vi "[ex ce] History of Script Variable.vi"() -> ()   [LabVIEW 2021]
doc: "<B>Variable Manager example</B>\n\nThe VI demonstrates details of how variable history works depending on its configuration. A variable is updated in CSE script and its history is read and indicated in parallel loop.\n\n::: CalcExpress Toolkit :::\nCopyright (c) 2000-2026 Konstantin Shifershteyn. All rights reserved."
uses:
  vi.lib/addons/CalcExpress/cetypes.llb/VarMan History Info.ctl
panel:
  in  "Value condition":T1 {"Range Max" format="%.3f"; "Range Min" format="%.3f"; "Delta" format="%.3f"}
  in  "Time condition":cluster{"Step, ms":i32, "Gate, ms":u32}
  in  "Condition selector":u16(ring)=1 caption="conditions example" items=["<custom condition>", "no conditions", "time step", "time step & out of range", "time step & time gate", "out of range", "within range"]
  out "graph":T2(graph) caption="The graph indicates history of the 'x' variable"
  out "history info":T3 caption="History info" {"oldest timestamp" format="%<%H:%M:%S%2u\n%d/%m/%Y>T"; "NewVals mode"."last read time" format="%<%H:%M:%S%2u\n%d/%m/%Y>T"; "newest timestamp" format="%<%H:%M:%S%2u\n%d/%m/%Y>T"}
  in  "History length":i32=100
  in  "script":string="if (x>=20) dx = -1;\nif (x<=0)  dx = 1;\nx += dx;\n"
  in  "stop":bool
  # "History Update Conditions"
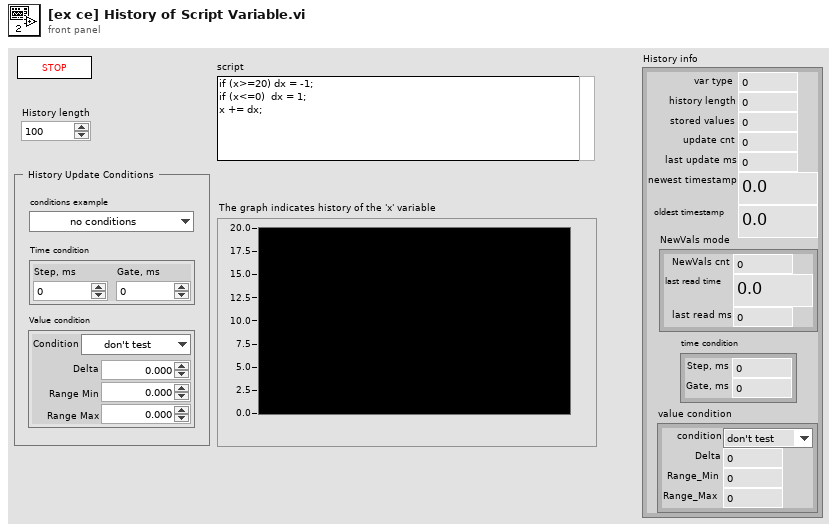
[diagram p1: front panel]
types:
  T1 = cluster{"Condition":enum32{"don't test", "changed", "abs deviation", "rel deviation", "out of range", "within range"}, "Delta":dbl, "Range Min":dbl, "Range Max":dbl}
  T2 = cluster{"history timestamps":dbl[], "history values":dbl[]}
  T3 = typedef "VarMan History Info.ctl" = cluster{"var type":u32, "history length":u32, "stored values":u32, "update cnt":u32, "last update ms":u32, "newest timestamp":dbl, "oldest timestamp":dbl, "NewVals mode":cluster{"NewVals cnt":u32, "last read time":dbl, "last read ms":u32}, "time condition":cluster{"Step, ms":u32, "Gate, ms":u32}, "value condition":cluster{"condition":enum32{"don't test", "changed", "abs deviation", "rel deviation", "out of range", "within range"}, "Delta":dbl, "Range_Min":dbl, "Range_Max":dbl}}
  T4 = cluster{"condition":enum32{"don't test", "changed", "abs deviation", "rel deviation", "out of range", "within range"}, "Delta":dbl, "Range_Min":dbl, "Range_Max":dbl}[]
  T5 = enum16{"create", "destroy", "set value", "get value"}
  T6 = enum32{"nop", "create", "destroy", "reset", "get info", "config"}
  T7 = typedef "VarMan Variable Context Handle.ctl" = i32
  T8 = cluster{"condition":enum32{"don't test", "changed", "abs deviation", "rel deviation", "out of range", "within range"}, "Delta":dbl, "Range_Min":dbl, "Range_Max":dbl}
  T9 = typedef "CSE Instance RefNum.ctl" = refnum<k1>
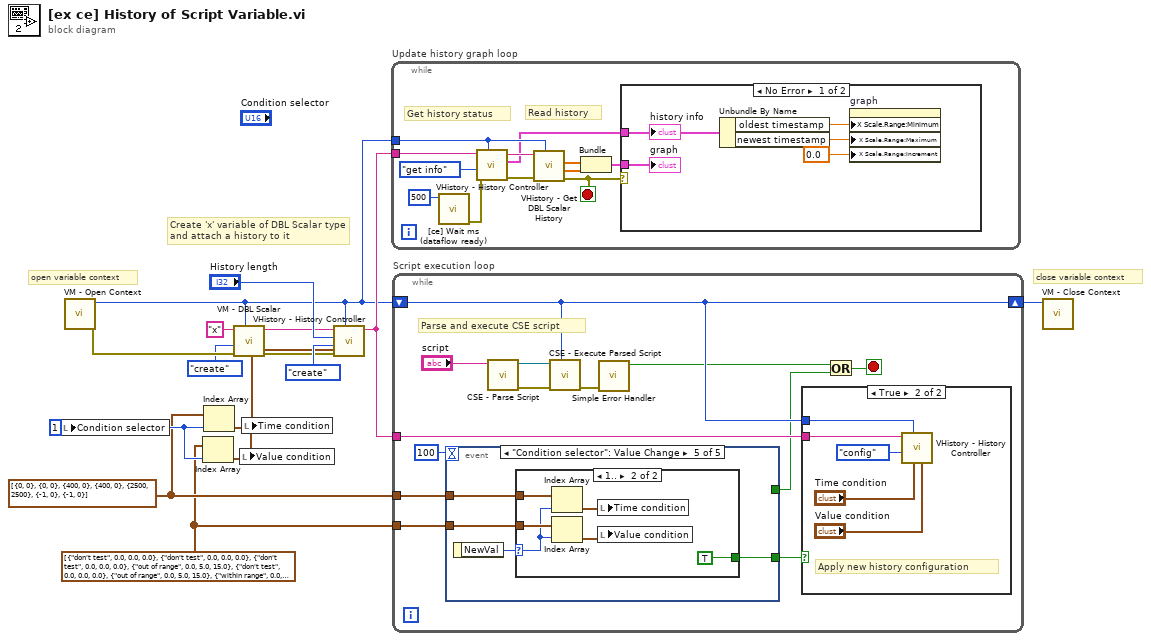
[diagram p0: block diagram]
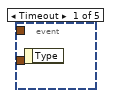
[diagram p2: hidden frame]
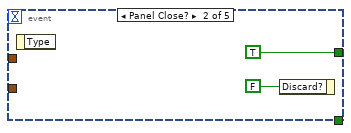
[diagram p3: hidden frame]
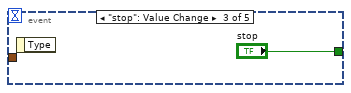
[diagram p4: hidden frame]
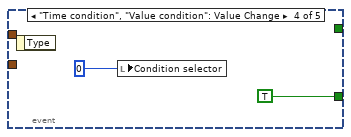
[diagram p5: hidden frame]
diagram:
  w5 = u16 1
  w1 = T4 [{"condition"=enum."don't test", "Delta"=0.0, "Range_Min"=0.0, "Range_Max"=0.0}, {"condition"=enum."don't test", "Delta"=0.0, "Range_Min"=0.0, "Range_Max"=0.0}, {"condition"=enum."don't test", "Delta"=0.0, "Range_Min"=0.0, "Range_Max"=0.0}, {"condition"=enum."out of range", "Delta"=0.0, "Range_Min"=5.0, "Range_Max"=15.0}, {"condition"=enum."don't test", "Delta"=0.0, "Range_Min"=0.0, "Range_Max"=0.0}, {"condition"=enum."out of range", "Delta"=0.0, "Range_Min"=5.0, "Range_Max"=15.0}, {"condition"=enum."within range", "Delta"=0.0, "Range_Min"=5.0, "Range_Max"=15.0}]
  w4 = cluster{"Step, ms":i32, "Gate, ms":u32}[] [{"Step, ms"=0, "Gate, ms"=0}, {"Step, ms"=0, "Gate, ms"=0}, {"Step, ms"=400, "Gate, ms"=0}, {"Step, ms"=400, "Gate, ms"=0}, {"Step, ms"=2500, "Gate, ms"=2500}, {"Step, ms"=-1, "Gate, ms"=0}, {"Step, ms"=-1, "Gate, ms"=0}]
  # "close variable context"
  # "Create 'x' variable of DBL Scalar type\nand attach a history to it"
  # "open variable context"
  n1 = local write "Condition selector"(w5) -> ()
  n2 = call "VM - Open Context.vi"() -> ("error out"=w11:errorcluster, "VC Handle out"=w6:T7)  [unwired: 9 in, 1 out]
  n3 = Index Array(array=w1, index=w5) -> (element=w2:T8)
  n4 = Index Array(array=w4, index=w5) -> (element=w3:cluster{"Step, ms":i32, "Gate, ms":u32})
  n5 = call "VM - DBL Scalar.vi"("VC Handle"=w6, "error in"=w11, "cmd"=T5."create", "name_spec"="x" ("name")) -> ("error out"=w12:errorcluster, "dup name_spec"=w8:string)  [unwired: 2 in, 4 out]
  n6 = local write "Value condition"(w2) -> ()
  n7 = local write "Time condition"(w3) -> ()
  n8 = call "VHistory - History Controller.vi"("value condition"=w2, "time conditions"=w3, "VC Handle"=w6, "error in"=w12, "cmd (nop:default)"=T6."create", "history length"="History length", "name_spec"=w8) -> ("dup name_spec"=w7:string)  [unwired: 1 in, 3 out]
  n9 = while "Update history graph loop" {
    tunnel: w6 -> [w21]
    tunnel: w7 -> [w22]
    stop <- w16 stop-if-true
    # "Read history"
    # "Get history status"
    n10 = call "[ce] Wait ms (dataflow ready).vi"("milliseconds to wait"=u32 500) -> ("error out"=w17:errorcluster)  [unwired: 4 in, 4 out]
    n11 = call "VHistory - History Controller.vi"("VC Handle"=w21, "error in"=w17, "cmd (nop:default)"=T6."get info", "name_spec"=w22) -> ("error out"=w24:errorcluster, "history info"=w20:T3, "dup name_spec"=w23:string)  [unwired: 4 in, 1 out]
    n12 = call "VHistory - Get DBL Scalar History.vi"("VC Handle"=w21, "error in"=w24, "name_spec"=w23) -> ("error out"=w16:errorcluster, "history"=w27:dbl[], "time stamps"=w25:dbl[])  [unwired: 4 in, 2 out]
    n13 = Bundle("time stamps"=w25, "history"=w27) -> (w26:cluster{"time stamps":dbl[], "history":dbl[]})  [unwired: 1 in]
    n14 = case shown="No Error" w16 {
      tunnel: w26 -> [w32 _]
      tunnel: w20 -> [w31 _]
      frame No Error {
        n15 = Unbundle By Name(w31) -> ("oldest timestamp"=w30:dbl, "newest timestamp"=w29:dbl)
        n16 = property on="graph" class="XYGraph (strict)"("X Scale.Range:Minimum"=w30, "X Scale.Range:Maximum"=w29, "X Scale.Range:Increment"=0.0 ("X Increment")) -> ()  [unwired: 2 in, 2 out]
        "graph" <- w32
        "history info" <- w31
      }
      frame Error {
      }
    }
  }
  n17 = while "Script execution loop" {
    tunnel: w1 -> [w37]
    tunnel: w4 -> [w38]
    tunnel: w7 -> [w42]
    shift-left: w6 -> [w41]
    shift-right: [w41] -> w15
    stop <- w33 stop-if-true
    # "Parse and execute CSE script"
    n18 = event shown="[4] \"Condition selector\": Value Change" {
      selector: _ -> [_ _ _ _ _]
      dyn-events: _ -> [_ _ _ _ _]
      timeout: 100 -> [_ _ _ _ _]
      tunnel: w38 -> [_ _ _ _ w54]
      tunnel: w37 -> [_ _ _ _ w53]
      tunnel: [_ _ _ TRUE w51] -> w36
      tunnel: [_ TRUE "stop" _ _] -> w35
      event Timeout {
        n19 = event-data() -> ()  [unwired: 1 in, 1 out]
      }
      event Panel Close? {
        n20 = event-data() -> ()  [unwired: 1 in, 1 out]
        n21 = event-data("Discard?"=FALSE) -> ()  [unwired: 1 in, 1 out]
      }
      event "stop": Value Change {
        n22 = event-data() -> ()  [unwired: 1 in, 1 out]
      }
      event "Time condition", "Value condition": Value Change {
        n23 = event-data() -> ()  [unwired: 1 in, 1 out]
        n24 = local write "Condition selector"(u16 0) -> ()
      }
      event "Condition selector": Value Change {
        n25 = event-data() -> ("NewVal"=w52:u16)  [unwired: 1 in]
        n26 = case shown="1.." w52 {
          selector: w52 -> [_ w56]
          tunnel: w54 -> [_ w58]
          tunnel: w53 -> [_ w57]
          tunnel: [_ TRUE] -> w51
          frame ..0 {
          }
          frame 1.. {
            n27 = Index Array(array=w58, index=w56) -> (element=w59:cluster{"Step, ms":i32, "Gate, ms":u32})
            n28 = Index Array(array=w57, index=w56) -> (element=w60:T8)
            n29 = local write "Time condition"(w59) -> ()
            n30 = local write "Value condition"(w60) -> ()
          }
        }
      }
    }
    n31 = call "CSE - Parse Script.vi"("Script"="script") -> ("error out"=w44:errorcluster, "CSE RefNum"=w43:T9)  [unwired: 6 in, 3 out]
    n32 = call "CSE - Execute Parsed Script.vi"("VC Handle"=w41, "error in"=w44, "CSE RefNum"=w43) -> ("error out"=w40:errorcluster)  [unwired: 4 in, 4 out]
    n33 = call <vilib>:"Simple Error Handler.vi"("error in (no error)"=w40) -> ("error?"=w34:bool)  [unwired: 4 in, 4 out]
    n34 = case shown="True" w36 {
      tunnel: w42 -> [_ w64]
      tunnel: w41 -> [_ w63]
      frame False {
      }
      frame True {
        # "Apply new history configuration"
        n35 = call "VHistory - History Controller.vi"("value condition"="Value condition", "time conditions"="Time condition", "VC Handle"=w63, "cmd (nop:default)"=T6."config", "name_spec"=w64) -> ()  [unwired: 3 in, 4 out]
      }
    }
    n36 = Or(x=w34, y=w35) -> (x .or. y?=w33:bool)
  }
  n37 = call "VM - Close Context.vi"("VC Handle"=w15) -> ()  [unwired: 9 in, 2 out]
